vi "CIVI Frequency Sweep Example.vi"() -> ()   [LabVIEW 2026]
doc: "Sweeps frequencies specified by Start, Stop and Step in kHz\nand records raw S-meter values.\nSets and reads back the mode once before the sweep.\nDisplays the XY graph after the loop finishes.\n\nThe panel STOP button ends the loop after the current iteration.\nOn normal completion or panel STOP, restores and verifies\nthe original frequency. The mode is not restored.\n\nAfter closing the connection, offers a CSV save dialog.\nCSV columns are frequency in kHz and raw S-meter value,\nwithout a header. Cancel skips saving.\n\nError recovery and automatic input validation are not implemented."
uses:
  c4f1cae7-0454-4689-a8a9-48d20d86a8a6.vi
  <vilib>/Utility/file.llb/Write Delimited Spreadsheet (DBL).vi
panel:
  in  "VISA Resource Name":refnum<visa-resource-name>="TCPIP0::127.0.0.1::5025::SOCKET"
  out "Mode":string
  out "Restore SCPI Error Code":i32
  out "Restored Frequency (Hz)":i32
  out "Restore Complete":string
  out "Original Frequency (Hz)":i32
  out "Frequency Sweep":cluster{dbl[], i32[]}(graph)
  in  "Abort":bool
  in  "Settling Time (ms)":u32
  in  "Step (kHz)":i32=1
  in  "Stop Frequency (kHz)":i32=800
  in  "Start Frequency (kHz)":i32=700
  out "SCPI Error Code":i32
  in  "Mode Setpint":string="AM"
  out "Operation Complete":string
  out "S Meter (raw)":i32
  out "error out":errorcluster
  out "Frequency (Hz)":i32
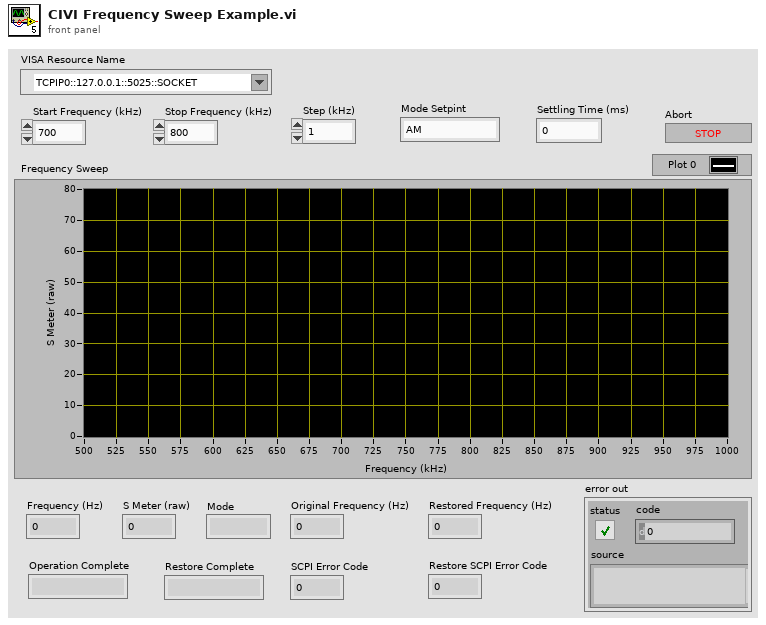
[diagram p1: front panel]
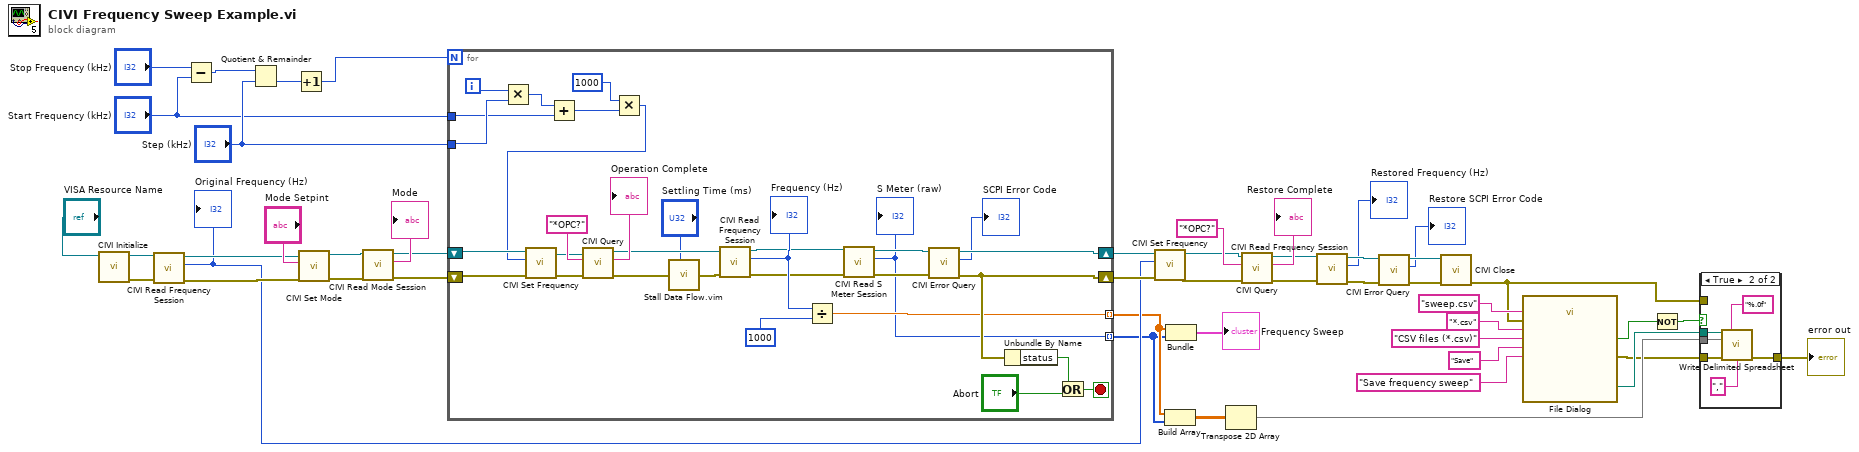
[diagram p0: block diagram]
diagram:
  n1 = call "CIVI Initialize.vi"("VISA Resource Name"="VISA Resource Name") -> ("error out"=w39:errorcluster, "VISA Session out"=w38:refnum<visa-resource-name>)  [unwired: 9 in]
  n2 = call "CIVI Read Frequency Session.vi"("error in"=w39, "VISA Session in"=w38) -> ("error out"=w36:errorcluster, "Frequency (Hz)"=w30:i32, "VISA Session out"=w37:refnum<visa-resource-name>)  [unwired: 7 in]
  "Original Frequency (Hz)" <- w30
  n3 = Subtract(x="Stop Frequency (kHz)", y="Start Frequency (kHz)") -> (x-y=w45:i32)
  n4 = Quotient & Remainder(x=w45, y="Step (kHz)") -> (floor(x/y)=w44:i32)  [unwired: 1 out]
  n5 = Increment(x=w44) -> (x+1=w43:i32)
  n6 = call "CIVI Set Mode.vi"("error in (no error)"=w36, "Mode"="Mode Setpint", "VISA Session in"=w37) -> ("error out"=w19:errorcluster, "VISA Session out"=w18:refnum<visa-resource-name>)  [unwired: 7 in]
  n7 = call "CIVI Read Mode Session.vi"("error in"=w19, "VISA Session in"=w18) -> ("error out"=w16:errorcluster, "Mode"=→"Mode":string, "VISA Session out"=w17:refnum<visa-resource-name>)  [unwired: 7 in]
  n8 = for {
    N: w43 -> [_]
    shift-right: [w76] -> w31
    shift-left: w17 -> [w72]
    shift-right: [w57] -> w32
    shift-left: w16 -> [w71]
    tunnel: "Step (kHz)" -> [w67]
    tunnel: "Start Frequency (kHz)" -> [w65]
    tunnel: [w52] -> w15 mode=indexing
    tunnel: [w51] -> w14 mode=indexing
    i -> [w68]
    stop <- w55 stop-if-true
    n9 = Multiply(x=w67, y=w68) -> (x*y=w66:i32)
    n10 = Add(x=w66, y=w65) -> (x+y=w64:i32)
    n11 = Multiply(x=1000, y=w64) -> (x*y=w62:i32)
    n12 = call "CIVI Set Frequency.vi"("error in (no error)"=w71, "Frequency Setpoint (Hz)"=w62, "VISA Session in"=w72) -> ("error out"=w70:errorcluster, "VISA Session out"=w69:refnum<visa-resource-name>)  [unwired: 7 in]
    n13 = call "CIVI Query.vi"("error in"=w70, "write buffer"="*OPC?", "VISA Session in"=w69) -> ("error out"=w60:errorcluster, "read buffer"=→"Operation Complete":string, "VISA Session out"=w77:refnum<visa-resource-name>)  [unwired: 6 in]
    n14 = call "Stall Data Flow.vim"("value in"=w60, "milliseconds to wait"="Settling Time (ms)") -> ("value out"=w59:errorcluster)  [unwired: 1 out]
    n15 = call "CIVI Read Frequency Session.vi"("error in"=w59, "VISA Session in"=w77) -> ("error out"=w50:errorcluster, "Frequency (Hz)"=w54:i32, "VISA Session out"=w49:refnum<visa-resource-name>)  [unwired: 7 in]
    "Frequency (Hz)" <- w54
    n16 = Divide(x=w54, y=1000) -> (x/y=w52:dbl)
    n17 = call "CIVI Read S Meter Session.vi"("error in"=w50, "VISA Session in"=w49) -> ("error out"=w74:errorcluster, "S Meter (raw)"=w51:i32, "VISA Session out"=w75:refnum<visa-resource-name>)  [unwired: 7 in]
    "S Meter (raw)" <- w51
    n18 = call "CIVI Error Query.vi"("error in"=w74, "VISA Session in"=w75) -> ("error out"=w57:errorcluster, "SCPI Error Code"=→"SCPI Error Code":i32, "VISA Session out"=w76:refnum<visa-resource-name>)  [unwired: 7 in]
    n19 = Unbundle By Name(w57) -> ("status"=w58:bool)
    n20 = Or(x=w58, y="Abort") -> (x .or. y?=w55:bool)
  }
  n21 = call "CIVI Set Frequency.vi"("error in (no error)"=w32, "Frequency Setpoint (Hz)"=w30, "VISA Session in"=w31) -> ("error out"=w33:errorcluster, "VISA Session out"=w34:refnum<visa-resource-name>)  [unwired: 7 in]
  n22 = Build Array(w15, w14) -> (w13:dbl[][])
  n23 = Bundle(w15, w14) -> (→"Frequency Sweep":cluster{dbl[], i32[]})  [unwired: 1 in]
  n24 = Transpose 2D Array(2D array=w13) -> (transposed array=w12:dbl[][])
  n25 = call "CIVI Query.vi"("error in"=w33, "write buffer"="*OPC?", "VISA Session in"=w34) -> ("error out"=w23:errorcluster, "read buffer"=→"Restore Complete":string, "VISA Session out"=w24:refnum<visa-resource-name>)  [unwired: 6 in]
  n26 = call "CIVI Read Frequency Session.vi"("error in"=w23, "VISA Session in"=w24) -> ("error out"=w28:errorcluster, "Frequency (Hz)"=→"Restored Frequency (Hz)":i32, "VISA Session out"=w27:refnum<visa-resource-name>)  [unwired: 7 in]
  n27 = call "CIVI Error Query.vi"("error in"=w28, "VISA Session in"=w27) -> ("error out"=w25:errorcluster, "SCPI Error Code"=→"Restore SCPI Error Code":i32, "VISA Session out"=w26:refnum<visa-resource-name>)  [unwired: 7 in]
  n28 = call "CIVI Close.vi"("error in"=w25, "VISA Session in"=w26) -> ("error out"=w1:errorcluster)  [unwired: 9 in]
  n29 = call "File Dialog"("prompt"="Save frequency sweep", "button label"="Save", "default name"="sweep.csv", "error in"=w1, "pattern (all files)"="*.csv", "pattern label"="CSV files (*.csv)") -> ("selected path"=w6:path, "cancelled"=w4:bool, "error out"=w2:errorcluster)  [unwired: 6 in, 1 out]
  n30 = Not(x=w4) -> (.not. x?=w5:bool)
  n31 = case shown="True" w5 {
    tunnel: w12 -> [_ w86]
    tunnel: w6 -> [_ w82]
    tunnel: w2 -> [_ w83]
    tunnel: [w80 w81] -> w3
    tunnel: w1 -> [w80 _]
    frame False {
    }
    frame True {
      n32 = call-poly <vilib>:"Write Delimited Spreadsheet.vi"("file path (dialog if empty)"=w82, "format (%.3f)"="%.0f", "2D data"=w86, "error in (no error)"=w83, "delimiter (\\t)"="," ("delimiter (\\t)")) -> ("error out"=w81:errorcluster)  [unwired: 9 in, 1 out]
    }
  }
  "error out" <- w3
